vi "to_json.vi"(8 "error in":errorcluster, 11 "exclude in":refnum<class "exclude.lvclass">) -> (0 "error out":errorcluster, 2 "json":string, 3 "exclude out":refnum<class "exclude.lvclass">, 4 "Not Default":bool)   [LabVIEW 2020, in "nominal types.lvlib" / "channelFilter.lvlib" / "exclude.lvclass"]
uses:
  exclude.lvclass
  exclude.lvclass/exclude.ctl
  d2a2ac13-5471-4191-9e88-4f0084fe2bd1.vi
  <vilib>/JDP Science/JSONtext/support/Format JSON Array Text.vi
  <vilib>/JDP Science/JSONtext/Variant to JSON Text.vi
  <vilib>/JDP Science/JSONtext/support/Format JSON Object.vi
  <vilib>/JDP Science/JSONtext/LVClass Serializer/JSONtext LVClass Serializer.lvclass
  <vilib>/JDP Science/JSONtext/JSONtext.lvlib
  filterTypes/filterTypes.lvclass
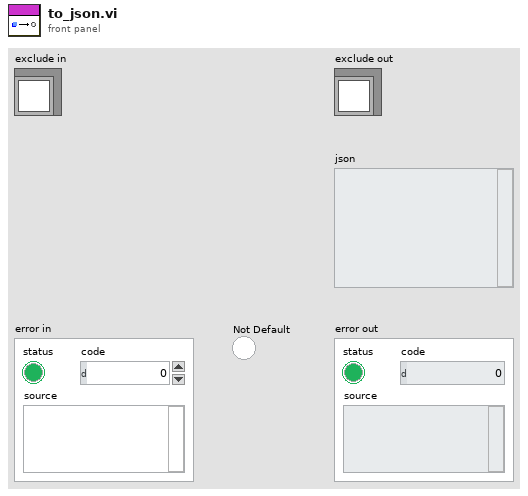
[diagram p1: front panel]
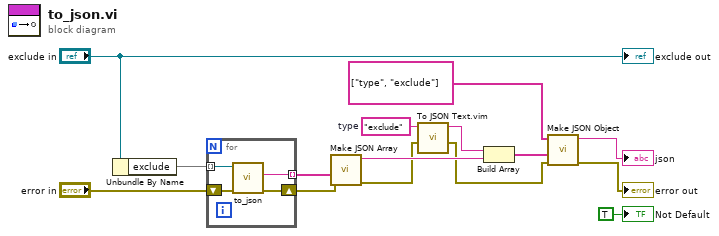
[diagram p0: block diagram]
diagram:
  w10 = "exclude"  # type
  n1 = Unbundle By Name("exclude in") -> ("exclude"=w14:set{refnum<class "filterTypes.lvclass">})
  n2 = for {
    tunnel: w14 -> [w17] mode=indexing
    tunnel: [w19] -> w12 mode=indexing
    shift-right: [w18] -> w11
    shift-left: "error in" -> [w16]
    n3 = call-dynamic "to_json.vi"("error in"=w16, "filterTypes in"=w17) -> ("error out"=w18:errorcluster, "json"=w19:string)  [unwired: 6 in, 2 out]
  }
  n4 = call <vilib>:"Make JSON Array.vi"("error in (no error)"=w11, "JSON Elements"=w12) -> ("error out"=w7:errorcluster, "<JSON>"=w8:string)  [unwired: 8 in]
  n5 = call "To JSON Text.vim"("error in (no error)"=w7, "Anything"=w10) -> ("error out"=w4:errorcluster, "<JSON>"=w9:string)  [unwired: 8 in]
  n6 = Build Array(w9, w8) -> (w6:string[])
  n7 = call <vilib>:"Make JSON Object.vi"("error in (no error)"=w4, "JSON Items"=w6, "Item Names"=string[] ["type", "exclude"]) -> ("error out"=→"error out":errorcluster, "<JSON>"=→"json":string)  [unwired: 7 in]
  "exclude out" <- "exclude in"
  "Not Default" <- TRUE ("Not Default")
